vi "Write Element.vi"(8 "error in":errorcluster, 10 "Element":refnum<class "IElement.lvclass">, 11 "Array in":refnum<class "Array.lvclass">) -> (0 "error out":errorcluster, 3 "Array out":refnum<class "Array.lvclass">)   [LabVIEW 2026, in "Array.lvclass"]
doc: "Data accessor."
uses:
  Array.lvclass
  Interfaces/IElement/IElement.lvclass
  Array.lvclass/Array.ctl
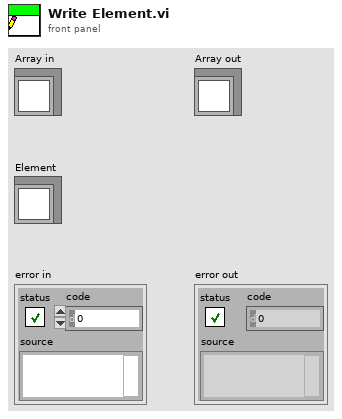
[diagram p1: front panel]
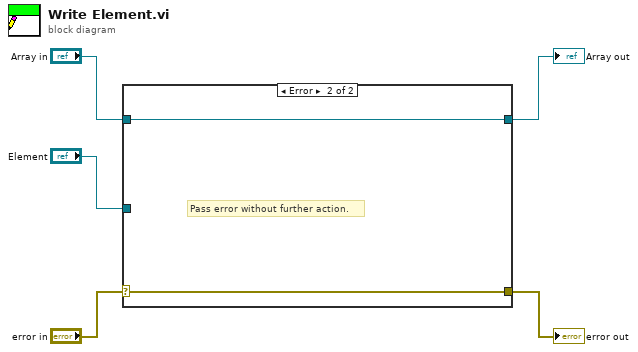
[diagram p0: block diagram]
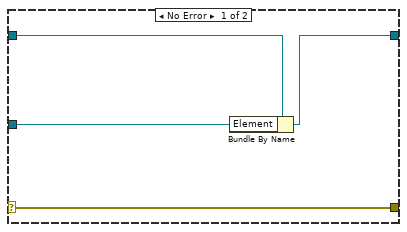
[diagram p2: hidden frame]
diagram:
  n1 = case shown="Error" "error in" {
    selector: "error in" -> [w9 w11]
    tunnel: [w9 w11] -> w4
    tunnel: [w7 w10] -> w2
    tunnel: "Array in" -> [w8 w10]
    tunnel: "Element" -> [w6 _]
    frame No Error {
      n2 = Bundle By Name(cluster=w8, "Element"=w6) -> (w7:refnum<class "Array.lvclass">)
    }
    frame Error {
      # "Pass error without further action."
    }
  }
  "error out" <- w4
  "Array out" <- w2
